vi "create_module_map.vi"(8 "error in (no error)":errorcluster, 10 "variable_info_in":T3) -> (0 "error out":errorcluster, 3 "IO_variable_map":T1[](array[typedef]))   [LabVIEW 2015, in "Scan Engine runtime.lvclass"]
uses:
  Scan Engine runtime.lvclass
  Custom Ctrls/Index Map.ctl
  <vilib>/NI/Tag Bus/tag/Data Type.ctl
  Custom Ctrls/IO_index_map.ctl
  <vilib>/NI/Tag Bus/tag/tag descriptor.lvclass
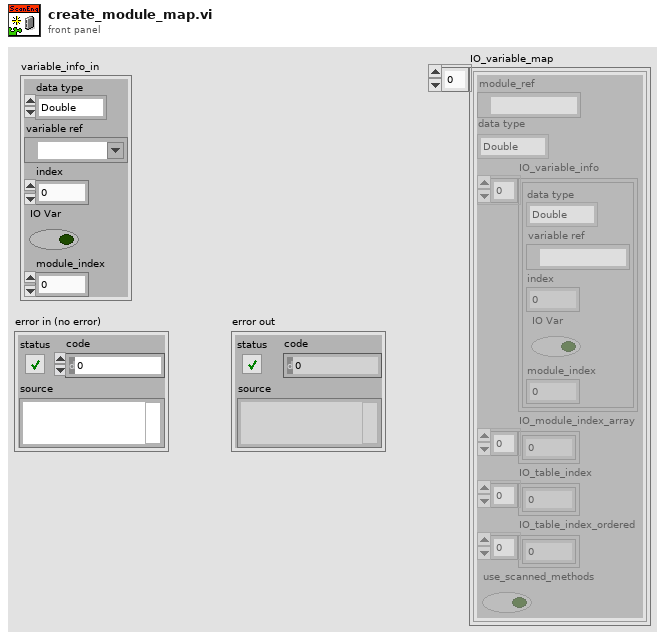
[diagram p1: front panel]
types:
  T1 = typedef "Scan Engine runtime.lvclass/IO_index_map.ctl" = cluster{"module_ref":refnum<k21>, "data type":T2, "IO_variable_info":T3[], "IO_module_index_array":i32[], "IO_table_index":i32[], "IO_table_index_ordered":i32[], "use_scanned_methods":bool}
  T2 = typedef "tag bus.lvlib/tag descriptor.lvclass/Data Type.ctl" = enum16{"Double", "Single", "I64", "I32", "I16", "I8", "U64", "U32", "U16", "U8", "Boolean", "String", "Array of Double", "Array of Single", "Array of I64", "Array of I32", "Array of I16", "Array of I8", "Array of U64", "Array of U32", "Array of U16", "Array of U8", "Array of Boolean", "Array of String"}
  T3 = typedef "Scan Engine runtime.lvclass/Index Map.ctl" = cluster{"data type":T2, "variable ref":refnum<k21>, "index":i32, "IO Var":bool, "module_index":i32}
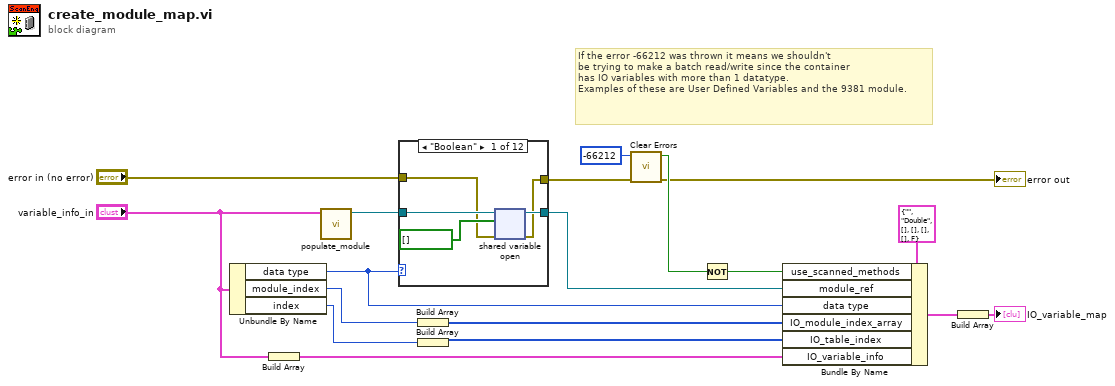
[diagram p0: block diagram]
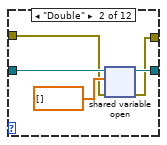
[diagram p2: hidden frame]
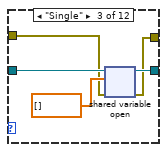
[diagram p3: hidden frame]
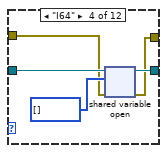
[diagram p4: hidden frame]
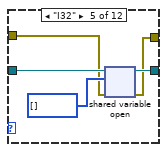
[diagram p5: hidden frame]
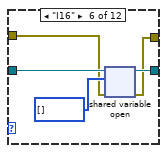
[diagram p6: hidden frame]
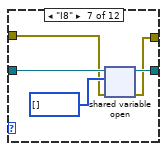
[diagram p7: hidden frame]
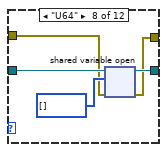
[diagram p8: hidden frame]
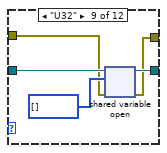
[diagram p9: hidden frame]
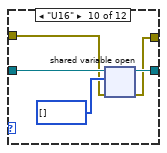
[diagram p10: hidden frame]
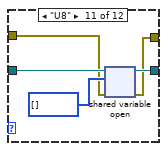
[diagram p11: hidden frame]
diagram:
  # "If the error -66212 was thrown it means we shouldn't\nbe trying to make a batch read/write since the container\nhas IO variables with more than 1 datatype.\nExamples of these are User Defined Variables and the 9381 module."
  n1 = Unbundle By Name("variable_info_in") -> ("data type"=w12:T2, "module_index"=w11:i32, "index"=w7:i32)
  n2 = Build Array("variable_info_in") -> (w9:T3[])
  n3 = call "populate_module.vi"("variable_info_in"="variable_info_in") -> ("Module"=w14:refnum<k21>)  [unwired: 10 in]
  n4 = case shown="\"Boolean\"" w12 {
    tunnel: [w21 w26 w31 w37 w41 w46 w51 w56 w61 w66 w71 w75] -> w13
    tunnel: w14 -> [w23 w28 w33 w38 w43 w48 w53 w58 w63 w68 w73 w75]
    tunnel: "error in (no error)" -> [w20 w25 w30 w35 w39 w44 w49 w54 w59 w64 w69 w74]
    tunnel: [w19 w24 w29 w34 w40 w45 w50 w55 w60 w65 w70 w74] -> w5
    frame "Boolean" {
      n5 = shared-variable-open(w23, w20, bool[] []) -> (w21:refnum<k21>, w19:errorcluster)
    }
    frame "Double" {
      n6 = shared-variable-open(w28, w25, dbl[] []) -> (w26:refnum<k21>, w24:errorcluster)
    }
    frame "Single" {
      n7 = shared-variable-open(w33, w30, sgl[] []) -> (w31:refnum<k21>, w29:errorcluster)
    }
    frame "I64" {
      n8 = shared-variable-open(w38, w35, i64[] []) -> (w37:refnum<k21>, w34:errorcluster)
    }
    frame "I32" {
      n9 = shared-variable-open(w43, w39, i32[] []) -> (w41:refnum<k21>, w40:errorcluster)
    }
    frame "I16" {
      n10 = shared-variable-open(w48, w44, i16[] []) -> (w46:refnum<k21>, w45:errorcluster)
    }
    frame "I8" {
      n11 = shared-variable-open(w53, w49, i8[] []) -> (w51:refnum<k21>, w50:errorcluster)
    }
    frame "U64" {
      n12 = shared-variable-open(w58, w54, u64[] []) -> (w56:refnum<k21>, w55:errorcluster)
    }
    frame "U32" {
      n13 = shared-variable-open(w63, w59, u32[] []) -> (w61:refnum<k21>, w60:errorcluster)
    }
    frame "U16" {
      n14 = shared-variable-open(w68, w64, u16[] []) -> (w66:refnum<k21>, w65:errorcluster)
    }
    frame "U8" {
      n15 = shared-variable-open(w73, w69, u8[] []) -> (w71:refnum<k21>, w70:errorcluster)
    }
    frame "String", Default {
    }
  }
  n16 = Build Array(w11) -> (w10:i32[])
  n17 = Build Array(w7) -> (w8:i32[])
  n18 = call <vilib>:"Clear Errors.vi"("error in (no error)"=w5, "specific error code to clear (0: all)"=-66212) -> ("error out"=→"error out":errorcluster, "specific error cleared?"=w3:bool)  [unwired: 4 in]
  n19 = Not(x=w3) -> (.not. x?=w2:bool)
  n20 = Bundle By Name(cluster=T1 {"module_ref"="", "data type"=enum."Double", "IO_variable_info"=[], "IO_module_index_array"=[], "IO_table_index"=[], "IO_table_index_ordered"=[], "use_scanned_methods"=FALSE} ("IO_variables_per_module"), "use_scanned_methods"=w2, "module_ref"=w13, "data type"=w12, "IO_module_index_array"=w10, "IO_table_index"=w8, "IO_variable_info"=w9) -> (w18:T1)
  n21 = Build Array(w18) -> (→"IO_variable_map":T1[])
